vi "Excel - Append Table Tests.vi"(8 "error in (no error)":errorcluster) -> (0 "error out":errorcluster)   [LabVIEW 2017]
uses:
  src/LabVIEW NPOI/MS-Excel/MS-Excel.lvclass
  C:/Users/Neo/Desktop/Dev_Tools_BR/LabVIEW_NPOI/src/LabVIEW NPOI/Document/Document.lvclass
  src/LabVIEW NPOI/Document/Append Table (string).vi
  src/LabVIEW NPOI/MS-Excel/Get Next Empty Cell.vi
  src/LabVIEW NPOI/Document/Append Table (double).vi
  <vilib>/addons/_JKI Toolkits/Caraya/classes/Assert/Assert Not Error.vi
  <vilib>/addons/_JKI Toolkits/Caraya/classes/Assert/Assert True.vi
  src/LabVIEW NPOI/Document/Document.lvclass
  <vilib>/addons/_JKI Toolkits/Caraya/classes/Test/Test.lvclass
  <vilib>/addons/_JKI Toolkits/Caraya/classes/Assert/Assert.lvclass
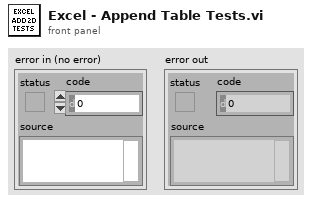
[diagram p1: front panel]
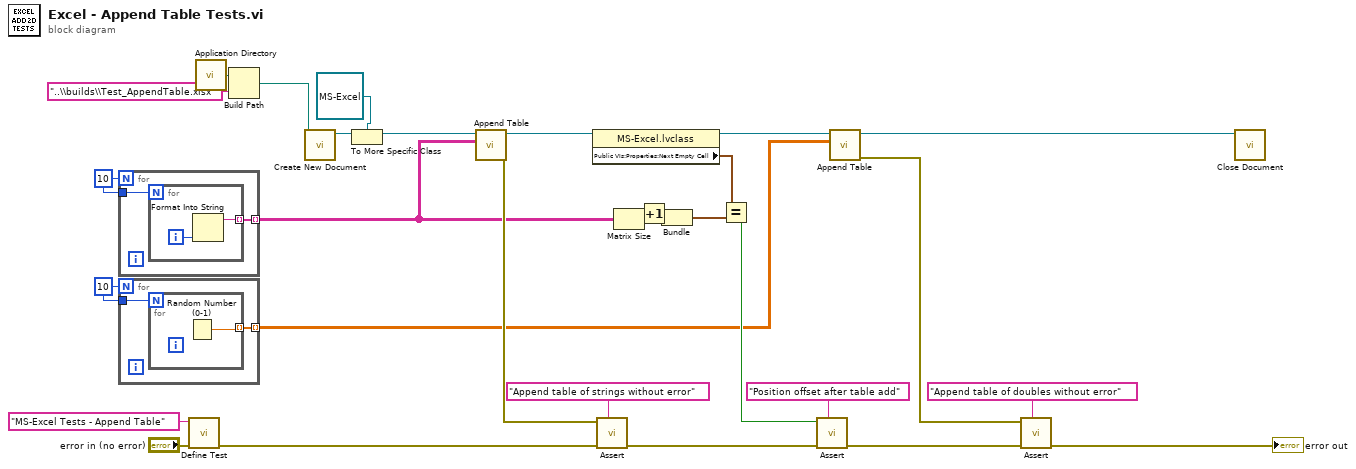
[diagram p0: block diagram]
diagram:
  w9 = 10
  w20 = 10
  n1 = for {
    N: w20 -> [_]
    tunnel: [w32] -> w12 mode=indexing
    tunnel: w20 -> [w31]
    n2 = for {
      N: w31 -> [_]
      tunnel: [w33] -> w32 mode=indexing
      i -> [w34]
      n3 = Format Into String(w34) -> (resulting string=w33:string)  [unwired: 3 in, 1 out]
    }
  }
  n4 = for {
    N: w9 -> [_]
    tunnel: [w36] -> w8 mode=indexing
    tunnel: w9 -> [w35]
    n5 = for {
      N: w35 -> [_]
      tunnel: [w37] -> w36 mode=indexing
      n6 = Random Number (0-1)() -> (number: 0 to 1=w37:dbl)
    }
  }
  n7 = call <vilib>:"Define Test.vi"("error in (no error)"="error in (no error)", "Label (VI Title)"="MS-Excel Tests - Append Table") -> ("error out"=w30:errorcluster)  [unwired: 9 in]
  n8 = call <vilib>:"Application Directory.vi"() -> ("Application Directory"=w24:path)
  n9 = Build Path(base path=w24, name or relative path="..\\builds\\Test_AppendTable.xlsx" ("string")) -> (appended path=w3:path)
  n10 = call "Create New Document.vi"("File Path"=w3) -> ("Document out"=w22:refnum<class "Document.lvclass">)  [unwired: 9 in, 1 out]
  n11 = To More Specific Class(target class=refnum<class "MS-Excel.lvclass"> refnum ("LabVIEW NPOI.lvlib:MS-Excel.lvclass"), reference=w22) -> (specific class reference=w2:refnum<class "MS-Excel.lvclass">)  [unwired: 1 in, 1 out]
  n12 = call-poly "Append Table.vi"("Table"=w12, "Document in"=w2) -> ("error out"=w13:errorcluster, "Document out"=w21:refnum<class "MS-Excel.lvclass">)  [unwired: 8 in]
  n13 = property class="MS-Excel.lvclass"(reference=w21) -> (reference out=w10:refnum<class "MS-Excel.lvclass">, "Public VIs:Properties:Next Empty Cell"=w19:cluster{"Row":i32, "Column":i32})  [unwired: 1 in, 1 out]
  n14 = call-poly <vilib>:"Assert.vi"("Label"="Append table of strings without error", "error in (no error)"=w30, "Not Error?"=w13) -> ("error out"=w28:errorcluster)  [unwired: 8 in]
  n15 = Matrix Size(0:w12) -> (1:w18:i32, 2:w17:i32)
  n16 = Increment(x=w18) -> (x+1=w14:i32)
  n17 = Bundle(w14, "matrix"=w17) -> (w16:cluster{i32, "matrix":i32})  [unwired: 1 in]
  n18 = Equal?(x=w19, y=w16) -> (x = y?=w15:bool)
  n19 = call-poly <vilib>:"Assert.vi"("Label"="Position offset after table add", "error in (no error)"=w28, "True?"=w15) -> ("error out"=w7:errorcluster)  [unwired: 8 in]
  n20 = call-poly "Append Table.vi"("Table"=w8, "Document in"=w10) -> ("error out"=w4:errorcluster, "Document out"=w11:refnum<class "MS-Excel.lvclass">)  [unwired: 8 in]
  n21 = call-poly <vilib>:"Assert.vi"("Label"="Append table of doubles without error", "error in (no error)"=w7, "Not Error?"=w4) -> ("error out"=→"error out":errorcluster)  [unwired: 8 in]
  n22 = call "Close Document.vi"("Document in"=w11) -> ()  [unwired: 10 in, 1 out]
